vi "Raw Subscriber from Refnum.vi"(3 "Raw Subscriber Refnum":T1 {"refnum" format="%.0x"}) -> (5 "Raw Subscriber U64":u64)   [LabVIEW 2021, in "Iceoryx.lvlib"]
uses:
  Iceoryx.lvlib
  Typedef/Raw Subscriber Refnum.ctl
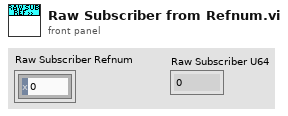
[diagram p1: front panel]
types:
  T1 = typedef "Iceoryx.lvlib/Raw Subscriber Refnum.ctl" = cluster{"refnum":u64, "Raw Sub":enum8{"rawsub"}}
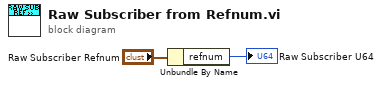
[diagram p0: block diagram]
diagram:
  n1 = Unbundle By Name("Raw Subscriber Refnum") -> ("refnum"=→"Raw Subscriber U64":u64)
